vi "FuncVI-Abs.vi"(5 "InstanceRef":T2, 9 "arg list":T1[](array[typedef]) {"num" format="%.2f"}) -> (0 "error out":bool, 3 "result":T1 {"num" format="%.2f"})   [LabVIEW 2021]
doc: "::: CalcExpress Toolkit :::\nCopyright (c) 2000-2026 Konstantin Shifershteyn. All rights reserved."
uses:
  cetypes.llb/CalcExpress Function Argument Info.ctl
  cetypes.llb/CalcExpress Instance RefNum.ctl
panel:
  in  "max arg num":i32=1
  in  "min arg num":i32=1
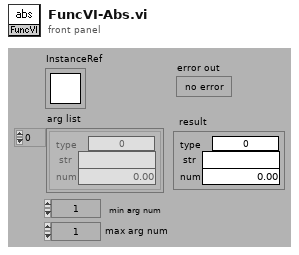
[diagram p1: front panel]
types:
  T1 = typedef "CalcExpress Function Argument Info.ctl" = cluster{"type":u32, "str":string, "num":dbl}
  T2 = typedef "CalcExpress Instance RefNum.ctl" = refnum<k1>
  T3 = enum16{"DBL scalar", "CDB scalar", "DBL array", "CDB array", "ERROR"}
  T4 = typedef "CalcExpress Data Type.ctl" = enum32{"String", "DBL Number", "identifier", "1D Array of DBL", "2D Array of DBL", "CDB Number", "1D Array of CDB", "2D Array of CDB", "1D Array of String", "2D Array of String", "Unknown data type"}
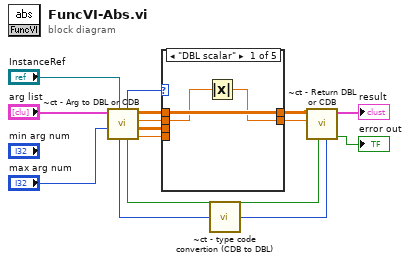
[diagram p0: block diagram]
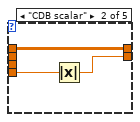
[diagram p2: hidden frame]
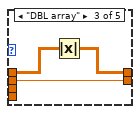
[diagram p3: hidden frame]
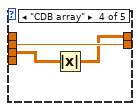
[diagram p4: hidden frame]
diagram:
  n1 = call "~ct - Arg to DBL or CDB.vi"("InstanceRef"="InstanceRef", "max args"="max arg num", "args list"="arg list") -> ("CDB"=w9:cdb, "2D CDB"=w10:cdb[][], "DBL"=w8:dbl, "2D DBL"=w7:dbl[][], "error out"=w11:bool, "category"=w4:T3, "arg type"=w3:T4)  [unwired: 2 in]
  n2 = case shown="\"DBL scalar\"" w4 {
    tunnel: w10 -> [_ _ _ w25 _]
    tunnel: w9 -> [_ w19 _ _ _]
    tunnel: w8 -> [w17 _ w24 w27 w28]
    tunnel: w7 -> [w18 w21 w23 _ w29]
    tunnel: [w18 w21 w22 w26 w29] -> w6
    tunnel: [w16 w20 w24 w27 w28] -> w5
    frame "DBL scalar" {
      n3 = Absolute Value(x=w17) -> (abs(x)=w16:dbl)
    }
    frame "CDB scalar" {
      n4 = Absolute Value(x=w19) -> (abs(x)=w20:dbl)
    }
    frame "DBL array" {
      n5 = Absolute Value(x=w23) -> (abs(x)=w22:dbl[][])
    }
    frame "CDB array" {
      n6 = Absolute Value(x=w25) -> (abs(x)=w26:dbl[][])
    }
    frame "ERROR" {
    }
  }
  n7 = call "~ct - type code convertion (CDB to DBL).vi"("type"=w3) -> ("type out"=w2:T4)  [unwired: 4 in]
  n8 = call "~ct - Return DBL or CDB.vi"("type"=w2, "error in"=w11, "DBL"=w5, "2D DBL"=w6) -> ("error out"=→"error out":bool, "result"=→"result":T1)  [unwired: 6 in]
